vi "set tp-pi2BPSK Enable.vi"(8 "error in (no error)":errorcluster, 10 "tp-pi2BPSK Enable?":bool, 11 "NR in":refnum<class "NR.lvclass">) -> (0 "error out":errorcluster, 3 "NR out":refnum<class "NR.lvclass">)   [LabVIEW 2023, in "ANRITSU Call Box.lvlib" / "NR.lvclass"]
uses:
  NR.lvclass
  NR.lvclass/NR.ctl
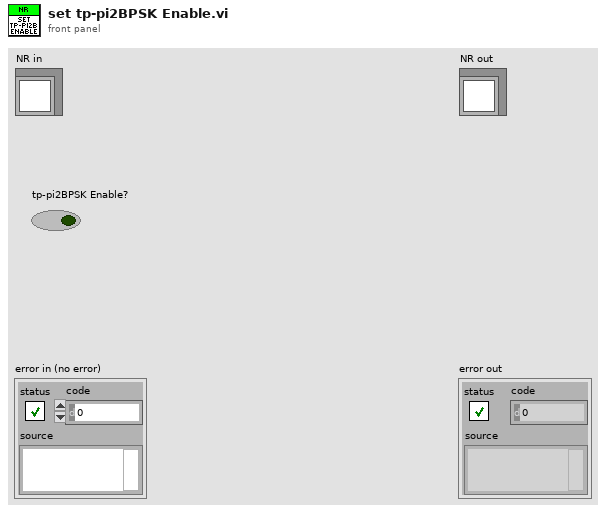
[diagram p1: front panel]
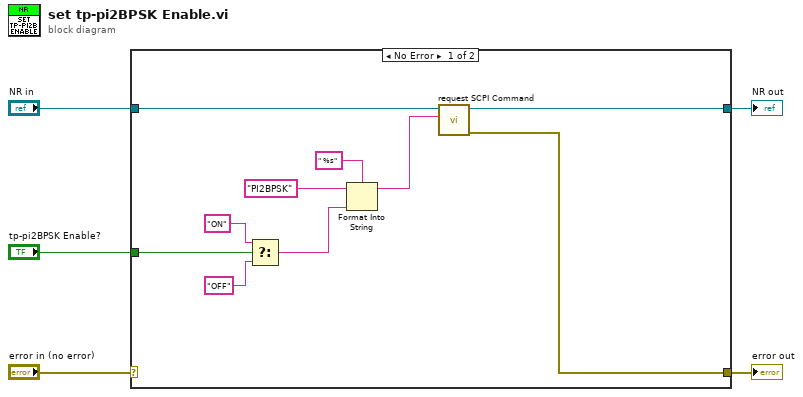
[diagram p0: block diagram]
diagram:
  n1 = case shown="No Error" "error in (no error)" {
    selector: "error in (no error)" -> [_ w17]
    tunnel: [w6 w17] -> w4
    tunnel: [w7 w16] -> w2
    tunnel: "NR in" -> [w9 w16]
    tunnel: "tp-pi2BPSK Enable?" -> [w13 _]
    frame No Error {
      n2 = Select(t="ON" ("initial string"), s=w13, f="OFF" ("initial string")) -> (s? t:f=w10:string)
      n3 = Format Into String(format string=" %s", initial string="PI2BPSK", w10) -> (resulting string=w8:string)  [unwired: 1 in, 1 out]
      n4 = call "request SCPI Command.vi"("SCPI Command"=w8, "NR in"=w9) -> ("error out"=w6:errorcluster, "NR out"=w7:refnum<class "NR.lvclass">)  [unwired: 8 in]
    }
    frame Error {
    }
  }
  "error out" <- w4
  "NR out" <- w2
